vi "读设备返回值 - WK.vi"(8 "错误输入（无错误）":errorcluster, 11 "VISA引用句柄输入":refnum<visa-resource-name>) -> (0 "错误输出":errorcluster, 1 "读取设备(n)":dbl, 2 "读取设备":string, 3 "VISA引用句柄输出":refnum<visa-resource-name>)   [LabVIEW 2017, in "UI-温度控制.lvlib"]
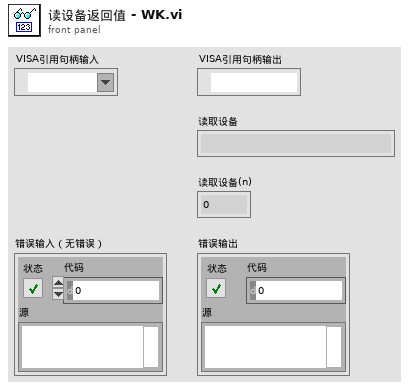
[diagram p1: front panel]
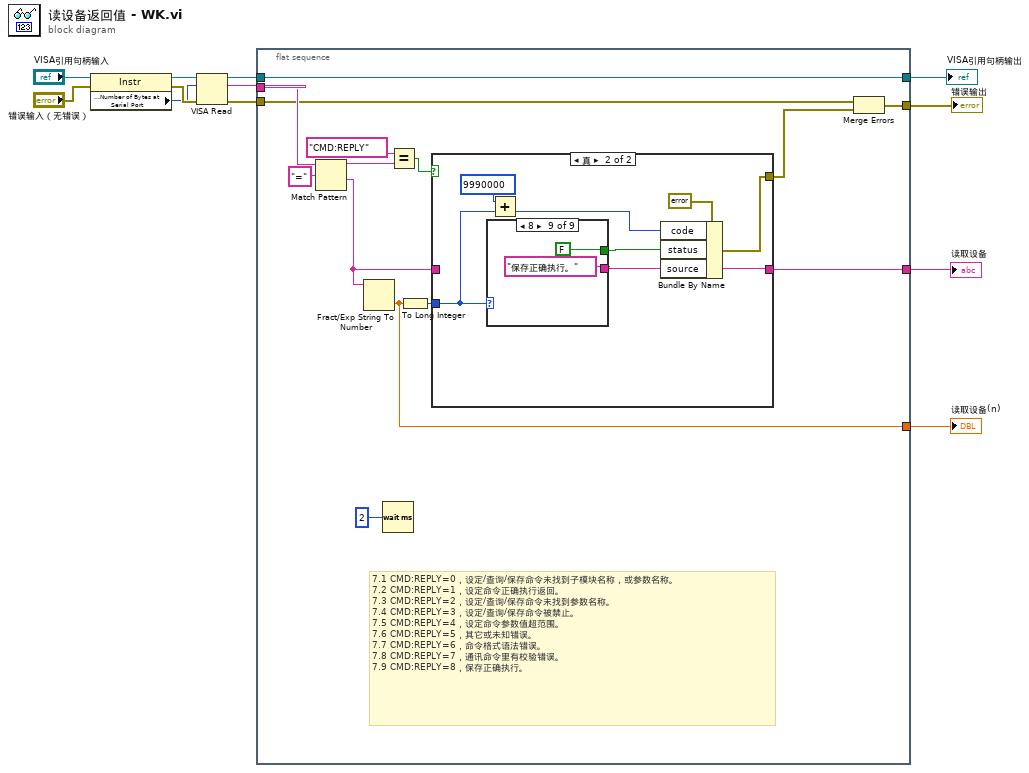
[diagram p0: block diagram]
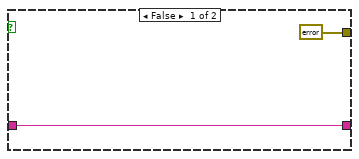
[diagram p2: hidden frame]
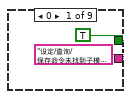
[diagram p3: hidden frame]
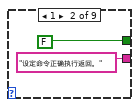
[diagram p4: hidden frame]
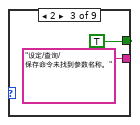
[diagram p5: hidden frame]
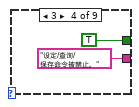
[diagram p6: hidden frame]
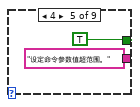
[diagram p7: hidden frame]
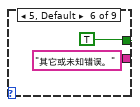
[diagram p8: hidden frame]
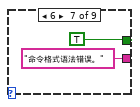
[diagram p9: hidden frame]
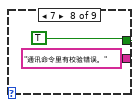
[diagram p10: hidden frame]
diagram:
  n1 = property class="Instr"(reference="VISA引用句柄输入", error in="错误输入（无错误）") -> (reference out=w3:refnum<visa-resource-name>, error out=w2:errorcluster, "Serial Settings:Number of Bytes at Serial Port"=w1:u32)
  n2 = VISA Read(VISA resource name=w3, byte count=w1, error in (no error)=w2) -> (VISA resource name out=w7:refnum<visa-resource-name>, read buffer=w8:string, error out=w6:errorcluster)  [unwired: 1 out]
  n3 = flat-sequence {
    tunnel: [w26] -> w11
    tunnel: w7 -> [w26]
    tunnel: [w15] -> w12
    tunnel: w6 -> [w14]
    tunnel: w8 -> [w24]
    tunnel: [w20] -> w9
    tunnel: [w17] -> w10
    frame #0 {
      # "7.1 CMD:REPLY=0，设定/查询/保存命令未找到子模块名称，或参数名称。\n7.2 CMD:REPLY=1，设定命令正确执行返回。\n7.3 CMD:REPLY=2，设定/查询/保存命令未找到参数名称。\n7.4 CMD:REPLY=3，设定/查询/保存命令被禁止。\n7.5 CMD:REPLY=4，设定命令参数值超范围。\n7.6 CMD:REPLY=5，其它或未知错误。\n7.7 CMD:REPLY=6，命令格式语法错误。\n7.8 CMD:REPLY=7，通讯命令里有校验错误。\n7.9 CMD:REPLY=8，保存正确执行。"
      n4 = Match Pattern(string=w24, regular expression="=" ("正则表达式")) -> (before substring=w21:string, after substring=w18:string)  [unwired: 1 in, 2 out]
      n5 = Fract/Exp String To Number(string=w18) -> (number=w17:dbl)  [unwired: 3 in, 1 out]
      n6 = Wait (ms)(milliseconds to wait=u32 2 ("等待时间（毫秒）")) -> ()  [unwired: 1 out]
      n7 = Equal?(x="CMD:REPLY", y=w21) -> (x = y?=w19:bool)
      n8 = To Long Integer(number=w17) -> (32bit integer=w16:i32)
      n9 = case shown="真" w19 {
        tunnel: w18 -> [w28 _]
        tunnel: [w28 w33] -> w20
        tunnel: w16 -> [_ w31]
        tunnel: [errorcluster {"status"=FALSE, "code"=0, "source"=""} ("错误常量") w32] -> w13
        frame False {
        }
        frame True {
          n10 = case shown="8" w31 {
            tunnel: ["设定/查询/保存命令未找到子模块名称，或参数名称。" ("read buffer") "设定命令正确执行返回。" ("read buffer") "设定/查询/保存命令未找到参数名称。" ("read buffer") "设定/查询/保存命令被禁止。" ("read buffer") "设定命令参数值超范围。" ("read buffer") "其它或未知错误。" ("read buffer") "命令格式语法错误。" ("read buffer") "通讯命令里有校验错误。" ("read buffer") "保存正确执行。" ("read buffer")] -> w33
            tunnel: [TRUE FALSE TRUE TRUE TRUE TRUE TRUE TRUE FALSE] -> w34
            frame 0 {
            }
            frame 1 {
            }
            frame 2 {
            }
            frame 3 {
            }
            frame 4 {
            }
            frame 5, Default {
            }
            frame 6 {
            }
            frame 7 {
            }
            frame 8 {
            }
          }
          n11 = Add(x=9990000, y=w31) -> (x+y=w30:i32)
          n12 = Bundle By Name(cluster=errorcluster {"status"=FALSE, "code"=0, "source"=""} ("错误常量"), "code"=w30, "status"=w34, "source"=w33) -> (w32:errorcluster)
        }
      }
      n13 = Merge Errors(w14, w13) -> (w15:errorcluster)
    }
  }
  "错误输出" <- w12
  "VISA引用句柄输出" <- w11
  "读取设备(n)" <- w10
  "读取设备" <- w9
